vi "box to conveyor.vi"(2 "error in (no error)":errorcluster, 3 "櫃子":i32) -> (0 "error out":errorcluster)   [LabVIEW 2019]
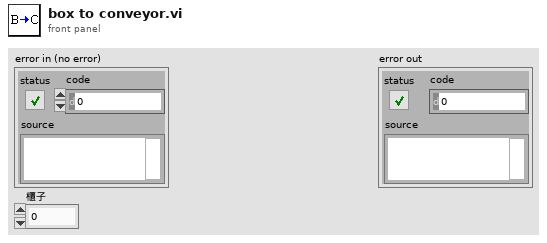
[diagram p1: front panel]
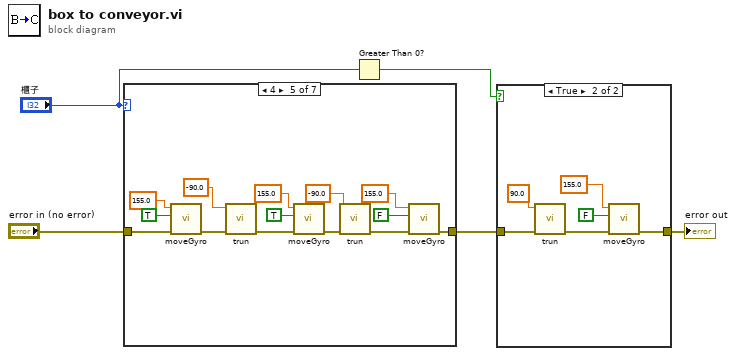
[diagram p0: block diagram]
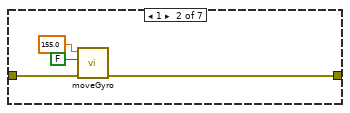
[diagram p4: hidden frame]
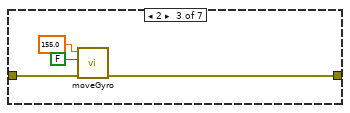
[diagram p5: hidden frame]
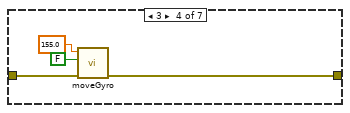
[diagram p6: hidden frame]
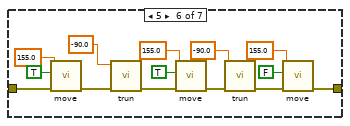
[diagram p7: hidden frame]
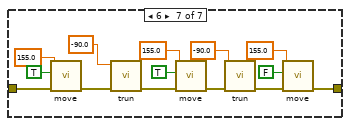
[diagram p8: hidden frame]
diagram:
  n1 = case shown="4" "櫃子" {
    tunnel: "error in (no error)" -> [w6 w9 w13 w17 w30 w46 w60]
    tunnel: [w6 w10 w14 w18 w22 w36 w50] -> w4
    frame 0, Default {
    }
    frame 1 {
      n2 = call "moveGyro.vi"("error in (no error)"=w9, "タは"=FALSE, "移動距離"=155.0) -> ("error out"=w10:errorcluster)  [unwired: 8 in]
    }
    frame 2 {
      n3 = call "moveGyro.vi"("error in (no error)"=w13, "タは"=FALSE, "移動距離"=155.0) -> ("error out"=w14:errorcluster)  [unwired: 8 in]
    }
    frame 3 {
      n4 = call "moveGyro.vi"("error in (no error)"=w17, "タは"=FALSE, "移動距離"=155.0) -> ("error out"=w18:errorcluster)  [unwired: 8 in]
    }
    frame 4 {
      n5 = call "moveGyro.vi"("error in (no error)"=w30, "タは"=TRUE, "移動距離"=155.0) -> ("error out"=w29:errorcluster)  [unwired: 8 in]
      n6 = call "trun.vi"("error in (no error)"=w29, "旋轉"=-90.0) -> ("error out"=w25:errorcluster)  [unwired: 9 in]
      n7 = call "moveGyro.vi"("error in (no error)"=w25, "タは"=TRUE, "移動距離"=155.0) -> ("error out"=w26:errorcluster)  [unwired: 8 in]
      n8 = call "trun.vi"("error in (no error)"=w26, "旋轉"=-90.0) -> ("error out"=w21:errorcluster)  [unwired: 9 in]
      n9 = call "moveGyro.vi"("error in (no error)"=w21, "タは"=FALSE, "移動距離"=155.0) -> ("error out"=w22:errorcluster)  [unwired: 8 in]
    }
    frame 5 {
      n10 = call "move.vi"("error in (no error)"=w46, "タは"=TRUE, "移動距離"=155.0) -> ("error out"=w43:errorcluster)  [unwired: 8 in]
      n11 = call "trun.vi"("error in (no error)"=w43, "旋轉"=-90.0) -> ("error out"=w41:errorcluster)  [unwired: 9 in]
      n12 = call "move.vi"("error in (no error)"=w41, "タは"=TRUE, "移動距離"=155.0) -> ("error out"=w38:errorcluster)  [unwired: 8 in]
      n13 = call "trun.vi"("error in (no error)"=w38, "旋轉"=-90.0) -> ("error out"=w35:errorcluster)  [unwired: 9 in]
      n14 = call "move.vi"("error in (no error)"=w35, "タは"=FALSE, "移動距離"=155.0) -> ("error out"=w36:errorcluster)  [unwired: 8 in]
    }
    frame 6 {
      n15 = call "move.vi"("error in (no error)"=w60, "タは"=TRUE, "移動距離"=155.0) -> ("error out"=w57:errorcluster)  [unwired: 8 in]
      n16 = call "trun.vi"("error in (no error)"=w57, "旋轉"=-90.0) -> ("error out"=w55:errorcluster)  [unwired: 9 in]
      n17 = call "move.vi"("error in (no error)"=w55, "タは"=TRUE, "移動距離"=155.0) -> ("error out"=w52:errorcluster)  [unwired: 8 in]
      n18 = call "trun.vi"("error in (no error)"=w52, "旋轉"=-90.0) -> ("error out"=w49:errorcluster)  [unwired: 9 in]
      n19 = call "move.vi"("error in (no error)"=w49, "タは"=FALSE, "移動距離"=155.0) -> ("error out"=w50:errorcluster)  [unwired: 8 in]
    }
  }
  n20 = Greater Than 0?(x="櫃子") -> (x > 0?=w2:bool)
  n21 = case shown="True" w2 {
    tunnel: w4 -> [w61 w67]
    tunnel: [w61 w63] -> w3
    frame False {
    }
    frame True {
      n22 = call "trun.vi"("error in (no error)"=w67, "旋轉"=90.0) -> ("error out"=w64:errorcluster)  [unwired: 9 in]
      n23 = call "moveGyro.vi"("error in (no error)"=w64, "タは"=FALSE, "移動距離"=155.0) -> ("error out"=w63:errorcluster)  [unwired: 8 in]
    }
  }
  "error out" <- w3
